vi "Hit_Check.vi"(0 "State":T1={"Tick"=0, "Phase"=0, "PhaseTicks"=0, "Level"=1, "Room"=0, "X10"=0, "Y10"=0, "VY10"=0, "Mode"=0, "Facing"=0, "Run"=0, "Vert"=0, "StandY"=0, "EntryX10"=0, "EntryY10"=0, "EntryMode"=0, "Lives"=4, "Score"=0, "NextLife"=10000, "KeyR"=0, "KeyB"=0, "KeyY"=0, "Torch"=FALSE, "FloorPhase"=0, "Dead"=FALSE, "LevelStart"=FALSE, "Quit"=FALSE, "Sound"=0, "Seed"=12345, "DemoStep"=0, "Tiles"=[], "World"=[], "Enemies"=[], "Highscores"=[], "Name"=[0, 0, 0], "Cursor"=0}, 11 "error in":errorcluster) -> (4 "Hit":bool, 15 "error out":errorcluster)   [LabVIEW 2020, in "GH_Engine.lvlib"]
doc: "Does an enemy touch Claude? Compares Claude's box (x 8..23, y 6..47 of his 32 x 48 picture) with the box of each enemy (spider, low snake that can be jumped over, skull)."
uses:
  GH_Engine.lvlib
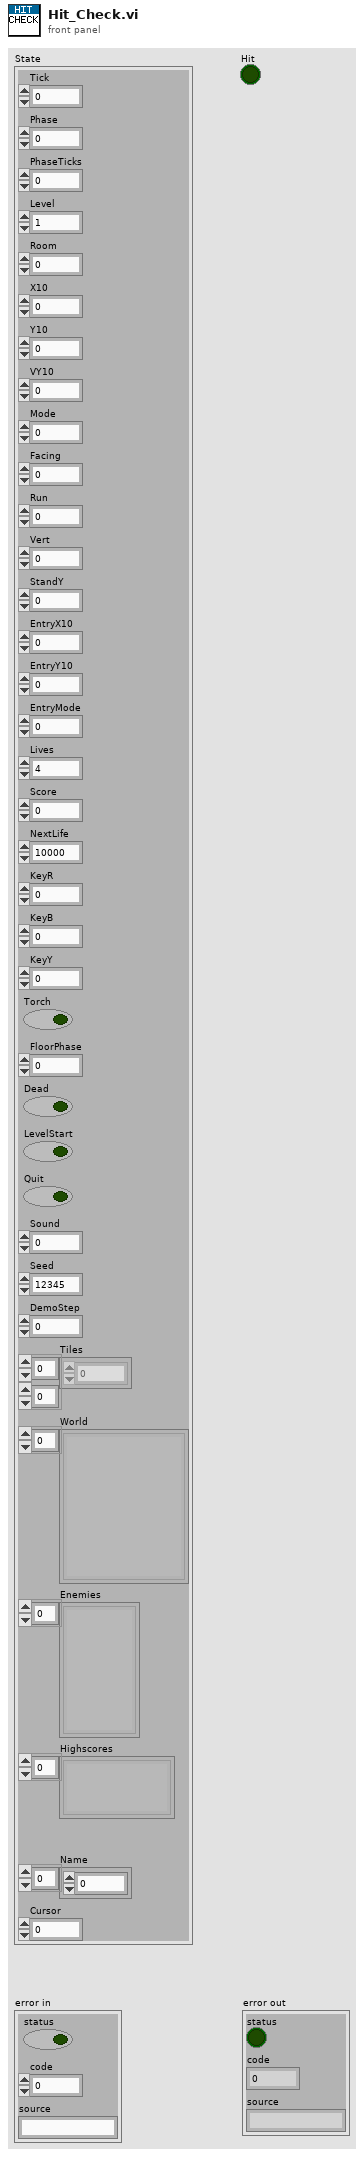
[diagram p1: front panel]
types:
  T1 = cluster{"Tick":u32, "Phase":i32, "PhaseTicks":i32, "Level":i32, "Room":i32, "X10":i32, "Y10":i32, "VY10":i32, "Mode":i32, "Facing":i32, "Run":i32, "Vert":i32, "StandY":i32, "EntryX10":i32, "EntryY10":i32, "EntryMode":i32, "Lives":i32, "Score":i32, "NextLife":i32, "KeyR":i32, "KeyB":i32, "KeyY":i32, "Torch":bool, "FloorPhase":i32, "Dead":bool, "LevelStart":bool, "Quit":bool, "Sound":i32, "Seed":u32, "DemoStep":i32, "Tiles":u8[][], "World":cluster{"ID":string, "Depth":i32, "Column":i32, "Tiles":u8[][]}[], "Enemies":cluster{"Kind":i32, "X10":i32, "Y10":i32, "Dir":i32, "Mode":i32}[], "Highscores":cluster{"Score":i32, "Name":string}[], "Name":i32[], "Cursor":i32}
  T2 = cluster{"Kind":i32, "X10":i32, "Y10":i32, "Dir":i32, "Mode":i32}[]
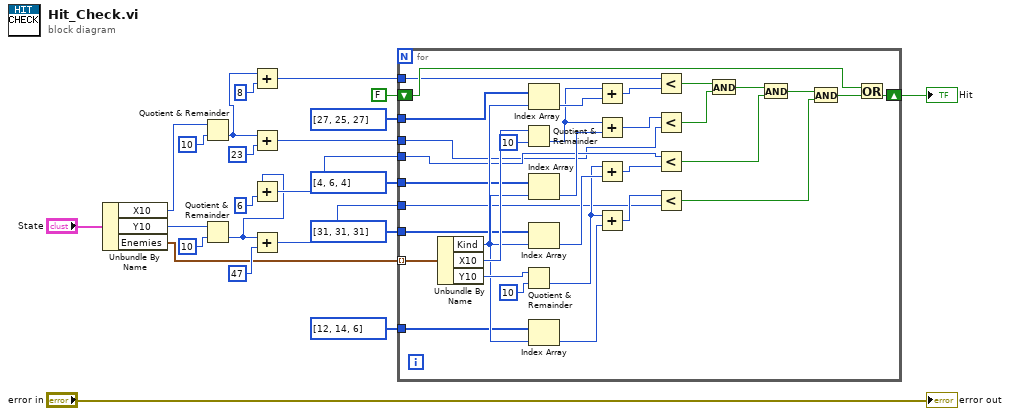
[diagram p0: block diagram]
diagram:
  n1 = Unbundle By Name("State") -> ("X10"=w3:i32, "Y10"=w4:i32, "Enemies"=w5:T2)
  n2 = Quotient & Remainder(x=w3, y=10) -> (floor(x/y)=w7:i32)  [unwired: 1 out]
  n3 = Quotient & Remainder(x=w4, y=10) -> (floor(x/y)=w9:i32)  [unwired: 1 out]
  n4 = Add(x=w7, y=8) -> (x+y=w11:i32)
  n5 = Add(x=w7, y=23) -> (x+y=w13:i32)
  n6 = Add(x=w9, y=6) -> (x+y=w15:i32)
  n7 = Add(x=w9, y=47) -> (x+y=w17:i32)
  n8 = for {
    tunnel: i32[] [4, 6, 4] ("Box left") -> [w29]
    tunnel: i32[] [27, 25, 27] ("Box right") -> [w30]
    tunnel: i32[] [12, 14, 6] ("Box top") -> [w31]
    tunnel: i32[] [31, 31, 31] ("Box bottom") -> [w32]
    shift-right: [w34] -> w23
    shift-left: FALSE -> [w33]
    tunnel: w5 -> [w24] mode=indexing
    tunnel: w11 -> [w25]
    tunnel: w13 -> [w26]
    tunnel: w15 -> [w27]
    tunnel: w17 -> [w28]
    n9 = Unbundle By Name(w24) -> ("Kind"=w35:i32, "X10"=w36:i32, "Y10"=w37:i32)
    n10 = Quotient & Remainder(x=w36, y=10) -> (floor(x/y)=w39:i32)  [unwired: 1 out]
    n11 = Quotient & Remainder(x=w37, y=10) -> (floor(x/y)=w41:i32)  [unwired: 1 out]
    n12 = Index Array(array=w30, index=w35) -> (element=w44:i32)
    n13 = Index Array(array=w29, index=w35) -> (element=w42:i32)
    n14 = Index Array(array=w32, index=w35) -> (element=w48:i32)
    n15 = Index Array(array=w31, index=w35) -> (element=w46:i32)
    n16 = Add(x=w39, y=w44) -> (x+y=w45:i32)
    n17 = Add(x=w39, y=w42) -> (x+y=w43:i32)
    n18 = Add(x=w41, y=w48) -> (x+y=w49:i32)
    n19 = Add(x=w41, y=w46) -> (x+y=w47:i32)
    n20 = Less?(x=w25, y=w45) -> (x < y?=w50:bool)
    n21 = Less?(x=w43, y=w26) -> (x < y?=w51:bool)
    n22 = Less?(x=w27, y=w49) -> (x < y?=w52:bool)
    n23 = Less?(x=w47, y=w28) -> (x < y?=w53:bool)
    n24 = And(x=w50, y=w51) -> (x .and. y?=w54:bool)
    n25 = And(x=w54, y=w52) -> (x .and. y?=w55:bool)
    n26 = And(x=w55, y=w53) -> (x .and. y?=w56:bool)
    n27 = Or(x=w33, y=w56) -> (x .or. y?=w34:bool)
  }
  "Hit" <- w23
  "error out" <- "error in"
